vi "to string.vi"(8 "error in":errorcluster, 11 "TDMS datalogger configuration in":refnum<class "TDMS datalogger configuration.lvclass">) -> (0 "error out":errorcluster, 1 "data":string, 2 "version":string, 3 "TDMS datalogger configuration out":refnum<class "TDMS datalogger configuration.lvclass">)   [LabVIEW 2015, in "TDMS datalogger configuration.lvclass"]
doc: "Provides an interface for saving a module configuration to a file or other serialized data source. It is recommended that all children of this class store data in two sets--data required for its own initialization, and any data required for parent initialization--and that each implementation uses the <b>Call Parent Method</b> primitive to serialize parent information."
uses:
  TDMS datalogger configuration.lvclass
  TDMS datalogger configuration.lvclass/TDMS datalogger configuration.ctl
  <vilib>/NI/Tag Bus Module Framework/module configuration/TBM module configuration.lvclass
  <vilib>/NI/Configuration Framework/serializable configuration/NISE_CEF_serializable configuration.lvclass
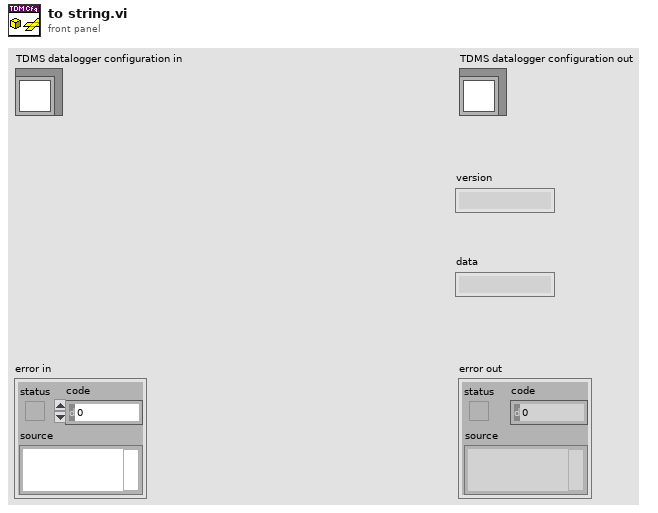
[diagram p1: front panel]
types:
  T1 = typedef "LogRotate.lvclass/options.ctl" = cluster{"max file size (bytes)":i64, "rotate count":u32, "max age (days)":dbl, "No archive dir":bool, "Archive dir":path}
  T2 = cluster{"channel":refnum<class "TBM channel.lvclass">}[]
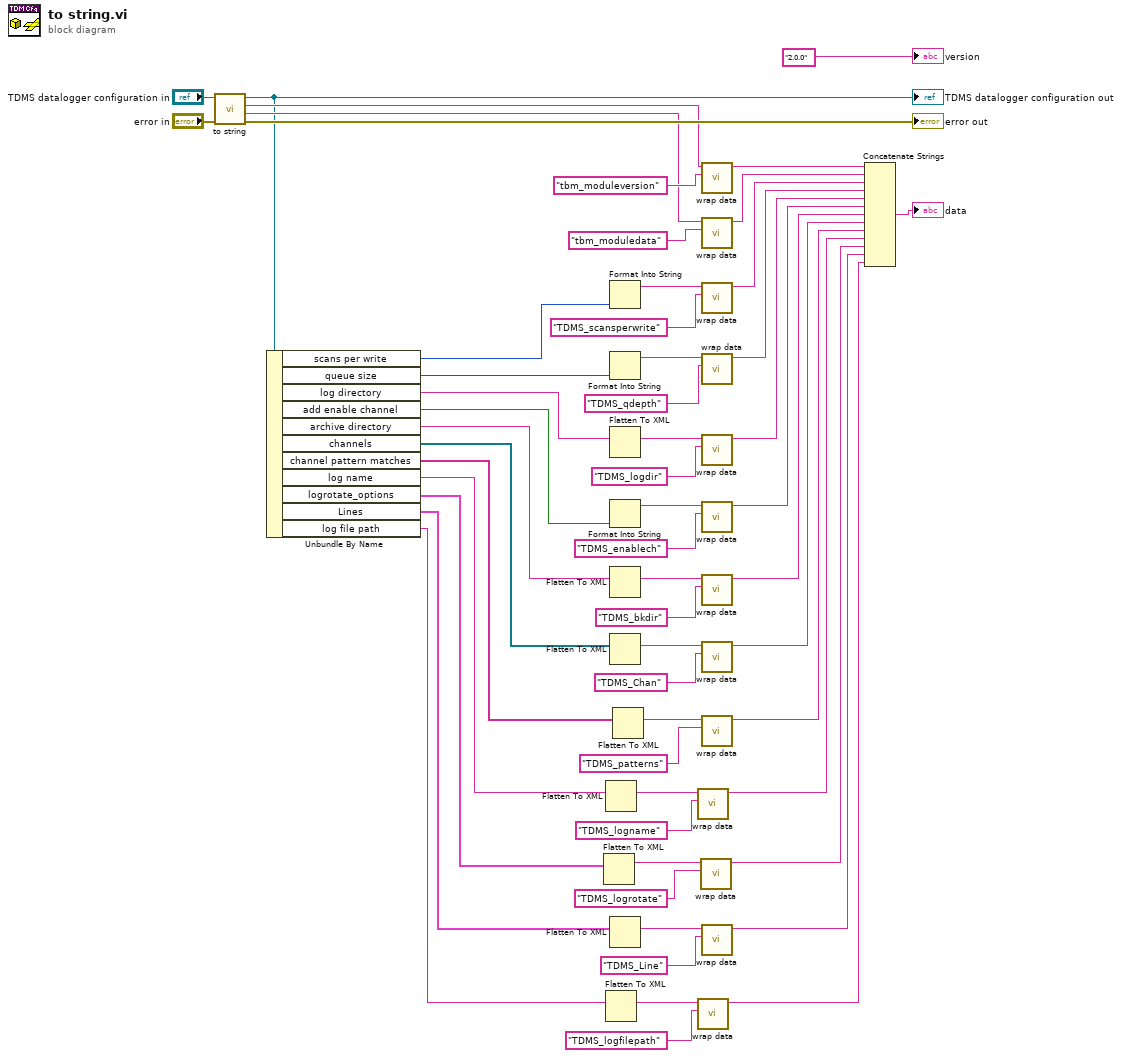
[diagram p0: block diagram]
diagram:
  n1 = call-parent "to string.vi"("error in"="error in", "module configuration in"="TDMS datalogger configuration in") -> ("error out"=→"error out":errorcluster, "data"=w50:string, "version"=w51:string, "module configuration out"=w46:refnum<class "TDMS datalogger configuration.lvclass">)  [unwired: 6 in]
  "TDMS datalogger configuration out" <- w46
  n2 = Unbundle By Name(w46) -> ("scans per write"=w42:u16, "queue size"=w43:u16, "log directory"=w18:string, "add enable channel"=w44:bool, "archive directory"=w17:string, "channels"=w45:refnum<class "TBM channel.lvclass">[], "channel pattern matches"=w23:string[], "log name"=w14:string, "logrotate_options"=w12:T1, "Lines"=w6:T2, "log file path"=w2:string)
  n3 = Flatten To XML(anything=w12) -> (xml string=w11:string)
  n4 = Flatten To XML(anything=w14) -> (xml string=w15:string)
  n5 = Flatten To XML(anything=w2) -> (xml string=w4:string)
  n6 = Format Into String(w42) -> (resulting string=w41:string)  [unwired: 3 in, 1 out]
  n7 = Format Into String(w43) -> (resulting string=w39:string)  [unwired: 3 in, 1 out]
  n8 = Flatten To XML(anything=w18) -> (xml string=w37:string)
  n9 = Format Into String(w44) -> (resulting string=w36:string)  [unwired: 3 in, 1 out]
  n10 = Flatten To XML(anything=w17) -> (xml string=w35:string)
  n11 = Flatten To XML(anything=w45) -> (xml string=w34:string)
  n12 = Flatten To XML(anything=w6) -> (xml string=w7:string)
  n13 = Flatten To XML(anything=w23) -> (xml string=w22:string)
  n14 = call <vilib>:"wrap data.vi"("identifier"="TDMS_logname" ("additional identifier"), "data to wrap"=w15) -> ("wrapped data"=w13:string)  [unwired: 9 in]
  n15 = call <vilib>:"wrap data.vi"("identifier"="TDMS_logfilepath" ("additional identifier"), "data to wrap"=w4) -> ("wrapped data"=w1:string)  [unwired: 9 in]
  n16 = call <vilib>:"wrap data.vi"("identifier"="TDMS_logrotate", "data to wrap"=w11) -> ("wrapped data"=w9:string)  [unwired: 9 in]
  n17 = call <vilib>:"wrap data.vi"("identifier"="tbm_moduleversion" ("additional identifier"), "data to wrap"=w51) -> ("wrapped data"=w49:string)  [unwired: 9 in]
  n18 = call <vilib>:"wrap data.vi"("identifier"="tbm_moduledata" ("additional identifier"), "data to wrap"=w50) -> ("wrapped data"=w47:string)  [unwired: 9 in]
  n19 = call <vilib>:"wrap data.vi"("identifier"="TDMS_scansperwrite" ("additional identifier"), "data to wrap"=w41) -> ("wrapped data"=w40:string)  [unwired: 9 in]
  n20 = call <vilib>:"wrap data.vi"("identifier"="TDMS_qdepth" ("additional identifier"), "data to wrap"=w39) -> ("wrapped data"=w38:string)  [unwired: 9 in]
  n21 = call <vilib>:"wrap data.vi"("identifier"="TDMS_logdir" ("additional identifier"), "data to wrap"=w37) -> ("wrapped data"=w33:string)  [unwired: 9 in]
  n22 = call <vilib>:"wrap data.vi"("identifier"="TDMS_enablech" ("additional identifier"), "data to wrap"=w36) -> ("wrapped data"=w32:string)  [unwired: 9 in]
  n23 = call <vilib>:"wrap data.vi"("identifier"="TDMS_bkdir" ("additional identifier"), "data to wrap"=w35) -> ("wrapped data"=w31:string)  [unwired: 9 in]
  n24 = call <vilib>:"wrap data.vi"("identifier"="TDMS_Chan" ("additional identifier"), "data to wrap"=w34) -> ("wrapped data"=w30:string)  [unwired: 9 in]
  n25 = call <vilib>:"wrap data.vi"("identifier"="TDMS_patterns", "data to wrap"=w22) -> ("wrapped data"=w20:string)  [unwired: 9 in]
  n26 = call <vilib>:"wrap data.vi"("identifier"="TDMS_Line" ("additional identifier"), "data to wrap"=w7) -> ("wrapped data"=w5:string)  [unwired: 9 in]
  n27 = Concatenate Strings(w49, w47, w40, w38, w33, w32, w31, w30, w20, w13, w9, w5, w1) -> (→"data":string)
  "version" <- "2.0.0" ("current version")
